vi "libssh2_session_last_errno.vi"(8 "error in (no error)":errorcluster, 11 "session":T1) -> (0 "error out":errorcluster, 2 "error code":i32)   [LabVIEW 2017, in "libssh2.lvlib"]
doc: "Get the last error code for a session."
uses:
  libssh2.lvlib
  Session Refnum.ctl
  Global Settings.vi
  Read Session Refnum.vi
  <vilib>/Utility/semaphor.llb/Acquire Semaphore.vi
  <vilib>/Utility/semaphor.llb/Release Semaphore.vi
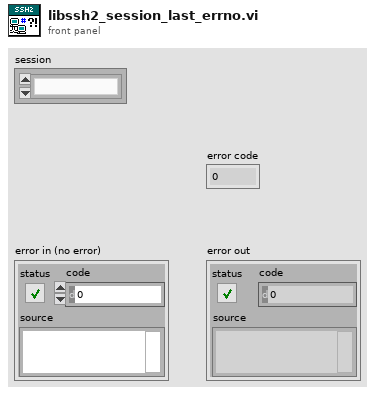
[diagram p1: front panel]
types:
  T1 = typedef "libssh2.lvlib/Session Refnum.ctl" = refnum<k1>
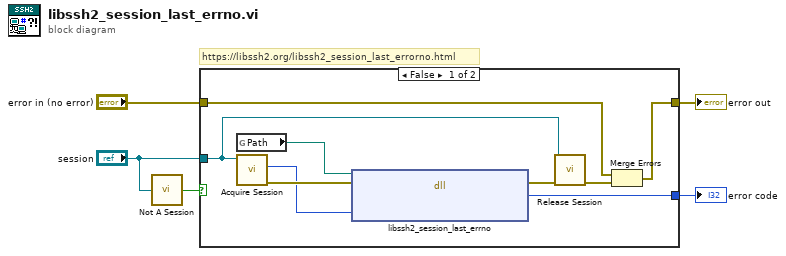
[diagram p0: block diagram]
diagram:
  # "https://libssh2.org/libssh2_session_last_errorno.html"
  n1 = call "Not A Session.vi"("session"="session") -> ("Not a Session?"=w1:bool)
  n2 = case shown="False" w1 {
    tunnel: [w10 w15] -> w5
    tunnel: [w14 _] -> w4
    tunnel: "error in (no error)" -> [w11 w15]
    tunnel: "session" -> [w6 _]
    frame False {
      n3 = global read "Global Settings.vi" "Path"() -> (w8:path)
      n4 = call "Acquire Session.vi"("session"=w6) -> ("error out"=w13:errorcluster, "LIBSSH2_SESSION*"=w12:u64)  [unwired: 8 in, 1 out]
      n5 = dll-call lib="?" fn="libssh2_session_last_errno"(path in=w8, error in=w13, "session"=w12) -> (error out=w9:errorcluster, "return value"=w14:i32)  [unwired: 2 in, 1 out]
      n6 = call "Release Session.vi"("error in (no error)"=w9, "session"=w6) -> ("error out"=w7:errorcluster)  [unwired: 9 in]
      n7 = Merge Errors(w11, w7) -> (w10:errorcluster)
    }
    frame True {
    }
  }
  "error out" <- w5
  "error code" <- w4
